vi "Built Chart.vi"(7 "Temperature":dbl) -> (3 "Chart":T1)   [LabVIEW 2021]
uses:
  Temperature Limits.vi
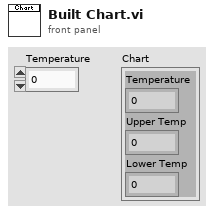
[diagram p1: front panel]
types:
  T1 = cluster{"Temperature":dbl, "Upper Temp":dbl, "Lower Temp":dbl}
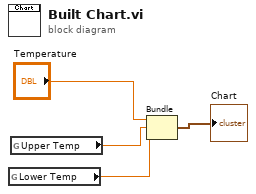
[diagram p0: block diagram]
diagram:
  n1 = global read "Temperature Limits.vi" "Lower Temp"() -> (w1:dbl)
  n2 = global read "Temperature Limits.vi" "Upper Temp"() -> (w2:dbl)
  n3 = Bundle("Temperature"="Temperature", "Upper Temp"=w2, "Lower Temp"=w1) -> (→"Chart":T1)  [unwired: 1 in]
